vi "work2_GetOrder.vi"() -> ()   [LabVIEW 2026]
panel:
  in  "Nb":i32
  in  "Burger":bool
  in  "Meal":bool
  in  "Stop":bool
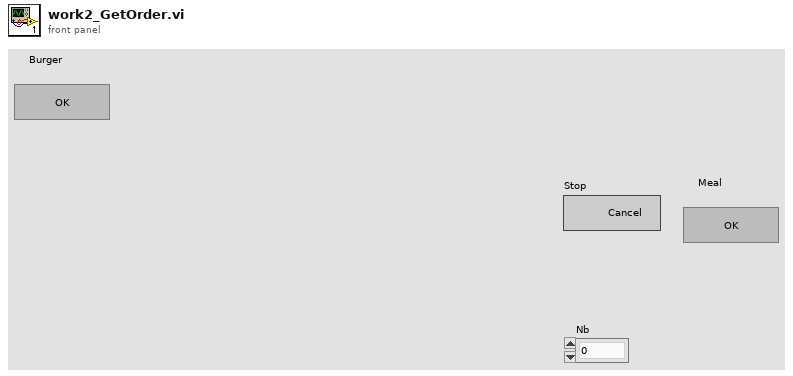
[diagram p1: front panel]
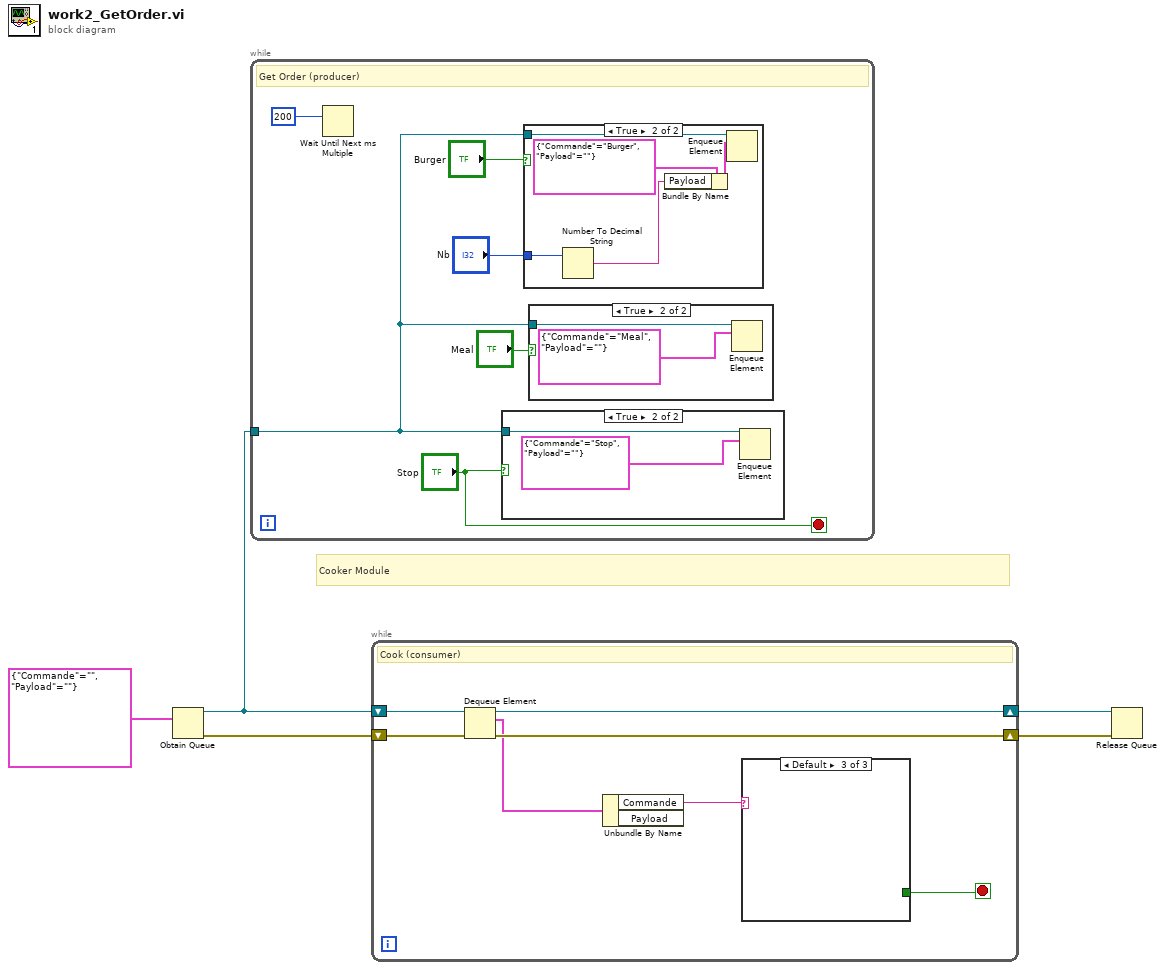
[diagram p0: block diagram]
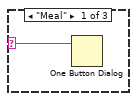
[diagram p5: hidden frame]
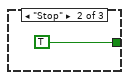
[diagram p6: hidden frame]
diagram:
  # "Cooker Module"
  n1 = Obtain Queue(element data type=cluster{"Commande":string, "Payload":string} {"Commande"="", "Payload"=""}) -> (queue out=w1:refnum<queue>, error out=w3:errorcluster)  [unwired: 4 in, 1 out]
  n2 = while {
    tunnel: w1 -> [w7]
    stop <- "Stop" stop-if-true
    # "Get Order (producer)"
    n3 = Wait Until Next ms Multiple(millisecond multiple=u32 200) -> ()  [unwired: 1 out]
    n4 = case shown="True" "Stop" {
      tunnel: w7 -> [_ w17]
      frame False {
      }
      frame True {
        n5 = Enqueue Element(queue=w17, element=cluster{"Commande":string, "Payload":string} {"Commande"="Stop", "Payload"=""}) -> ()  [unwired: 2 in, 3 out]
      }
    }
    n6 = case shown="True" "Burger" {
      tunnel: w7 -> [_ w16]
      tunnel: "Nb" -> [_ w12]
      frame False {
      }
      frame True {
        n7 = Number To Decimal String(number=w12) -> (decimal integer string=w13:string)  [unwired: 1 in]
        n8 = Bundle By Name(cluster=cluster{"Commande":string, "Payload":string} {"Commande"="Burger", "Payload"=""}, "Payload"=w13) -> (w14:cluster{"Commande":string, "Payload":string})
        n9 = Enqueue Element(queue=w16, element=w14) -> ()  [unwired: 2 in, 3 out]
      }
    }
    n10 = case shown="True" "Meal" {
      tunnel: w7 -> [_ w19]
      frame False {
      }
      frame True {
        n11 = Enqueue Element(queue=w19, element=cluster{"Commande":string, "Payload":string} {"Commande"="Meal", "Payload"=""}) -> ()  [unwired: 2 in, 3 out]
      }
    }
  }
  n12 = while {
    shift-right: [w26] -> w5
    shift-left: w1 -> [w27]
    shift-right: [w25] -> w4
    shift-left: w3 -> [w24]
    stop <- w21 stop-if-true
    # "Cook (consumer)"
    n13 = Dequeue Element(queue=w27, error in (no error)=w24) -> (queue out=w26:refnum<queue>, element=w23:cluster{"Commande":string, "Payload":string}, error out=w25:errorcluster)  [unwired: 1 in, 1 out]
    n14 = Unbundle By Name(w23) -> ("Commande"=w22:string)  [unwired: 1 out]
    n15 = case shown="Default" w22 {
      selector: w22 -> [w28 _ _]
      tunnel: [_ TRUE _] -> w21
      frame "Meal" {
        n16 = One Button Dialog(message=w28) -> ()  [unwired: 1 in, 1 out]
      }
      frame "Stop" {
      }
      frame Default {
      }
    }
  }
  n17 = Release Queue(queue=w5, error in (no error)=w4) -> ()  [unwired: 1 in, 3 out]
